vi "To CSV File.vi"(8 "error in (no error)":errorcluster, 9 "Path":path, 10 "engine configuration":refnum<class "engine configuration.lvclass">, 11 "PID Module editor node in":refnum<class "PID Module editor node.lvclass">) -> (0 "error out":errorcluster, 3 "PID Module editor node out":refnum<class "PID Module editor node.lvclass">)   [LabVIEW 2015, in "PID Module editor node.lvclass"]
uses:
  PID Module editor node.lvclass
  <vilib>/NI/Module Execution Interface/Engine Configuration/engine configuration.lvclass
  module/configuration/PID Module configuration.lvclass
  <vilib>/NI/Configuration Framework/serializable configuration/NISE_CEF_serializable configuration.lvclass/NISE_CEF_serializable configuration.ctl
  module/configuration/PID Module configuration.lvclass/PID Module configuration.ctl
  <vilib>/Utility/LVClass/Get LV Class Name.vi
  <vilib>/NI/Configuration Framework/error generator/NISE_error generator.vi
  <vilib>/NI/Tag Bus Module Framework/channel/TBM channel.lvclass
  <vilib>/NI/Configuration Framework/serializable configuration/NISE_CEF_serializable configuration.lvclass
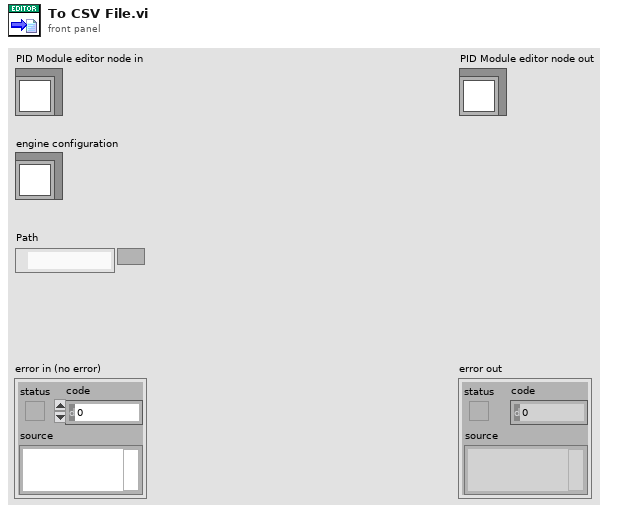
[diagram p1: front panel]
types:
  T1 = typedef "PID Module configuration.lvclass/Line.ctl" = cluster{"PID ID":string, "Setpoint":refnum<class "TBM channel.lvclass">, "Variable":refnum<class "TBM channel.lvclass">, "Output":refnum<class "TBM channel.lvclass">, "Output High":refnum<class "TBM channel.lvclass">, "Output Low":refnum<class "TBM channel.lvclass">, "P":refnum<class "TBM channel.lvclass">, "I":refnum<class "TBM channel.lvclass">, "D":refnum<class "TBM channel.lvclass">}
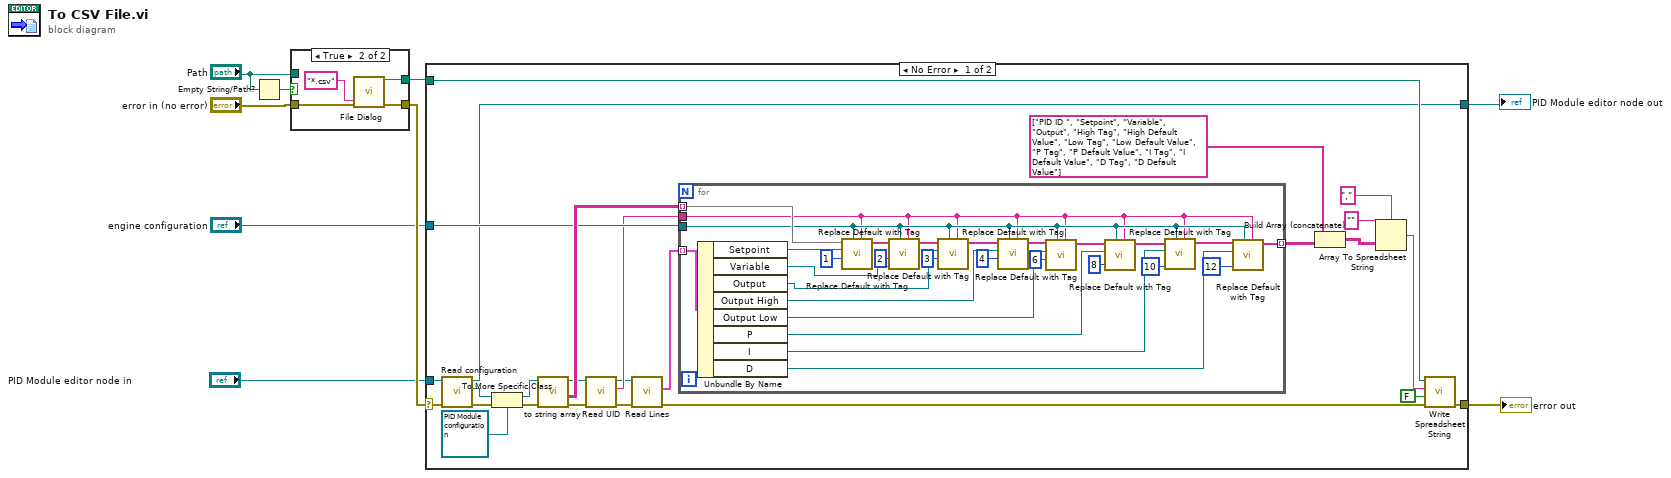
[diagram p0: block diagram]
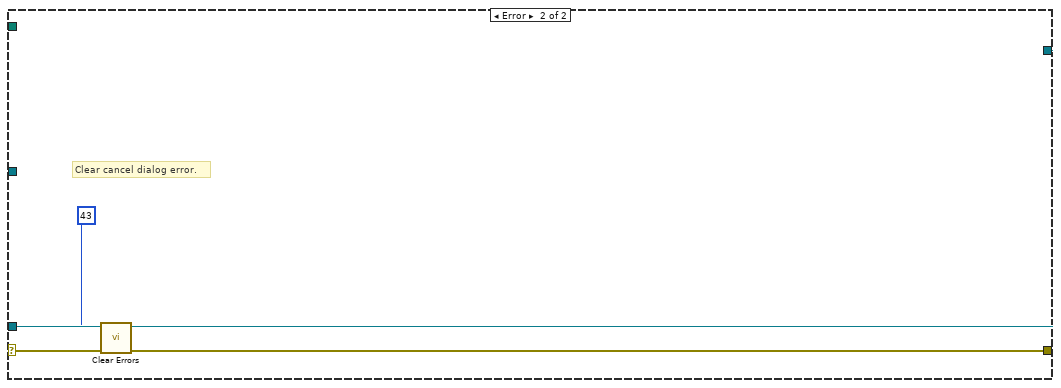
[diagram p3: hidden frame]
diagram:
  n1 = Empty String/Path?(string/path="Path") -> (empty?=w9:bool)
  n2 = case shown="True" w9 {
    tunnel: "error in (no error)" -> [w10 w14]
    tunnel: [w10 w13] -> w7
    tunnel: [w11 w12] -> w8
    tunnel: "Path" -> [w11 _]
    frame False {
    }
    frame True {
      n3 = call "File Dialog"("error in"=w14, "pattern (all files)"="*.csv") -> ("selected path"=w12:path, "error out"=w13:errorcluster)  [unwired: 10 in, 2 out]
    }
  }
  n4 = case shown="No Error" w7 {
    selector: w7 -> [w28 w72]
    tunnel: [w39 w71] -> w2
    tunnel: [w27 w73] -> w1
    tunnel: "PID Module editor node in" -> [w29 w73]
    tunnel: w8 -> [w35 _]
    tunnel: "engine configuration" -> [w32 _]
    frame No Error {
      n5 = call-dynamic "Read configuration.vi"("error in"=w28, "PID Module editor node in"=w29) -> ("error out"=w26:errorcluster, "configuration"=w25:refnum<class "NISE_CEF_serializable configuration.lvclass">, "PID Module editor node out"=w27:refnum<class "PID Module editor node.lvclass">)  [unwired: 7 in]
      n6 = To More Specific Class(target class=refnum<class "PID Module configuration.lvclass"> refnum ("tag bus configurable plugin module configuration"), reference=w25, error in=w26) -> (specific class reference=w41:refnum<class "PID Module configuration.lvclass">, error out=w40:errorcluster)
      n7 = call-dynamic "to string array.vi"("error in (no error)"=w40, "PID Module configuration in"=w41) -> ("error out"=w23:errorcluster, "Array"=w34:string[][], "PID Module configuration out"=w24:refnum<class "PID Module configuration.lvclass">)  [unwired: 6 in, 1 out]
      n8 = call <vilib>:"Read UID.vi"("error in"=w23, "configuration in"=w24) -> ("error out"=w21:errorcluster, "instance id"=w31:string, "configuration out"=w18:refnum<class "PID Module configuration.lvclass">)  [unwired: 7 in]
      n9 = call "Read Lines.vi"("error in (no error)"=w21, "PID Module configuration in"=w18) -> ("error out"=w20:errorcluster, "Lines"=w19:T1[])  [unwired: 7 in, 1 out]
      n10 = for {
        tunnel: w34 -> [w68] mode=indexing
        tunnel: [w56] -> w33 mode=indexing
        tunnel: w19 -> [w69] mode=indexing
        tunnel: w32 -> [w53]
        tunnel: w31 -> [w42]
        n11 = Unbundle By Name(w69) -> ("Setpoint"=w64:refnum<class "TBM channel.lvclass">, "Variable"=w63:refnum<class "TBM channel.lvclass">, "Output"=w62:refnum<class "TBM channel.lvclass">, "Output High"=w61:refnum<class "TBM channel.lvclass">, "Output Low"=w60:refnum<class "TBM channel.lvclass">, "P"=w59:refnum<class "TBM channel.lvclass">, "I"=w55:refnum<class "TBM channel.lvclass">, "D"=w54:refnum<class "TBM channel.lvclass">)
        n12 = call "Replace Default with Tag.vi"("instance id"=w42, "engine configuration in"=w53, "Channel Index"=1, "Channel"=w64, "Array in"=w68) -> ("Array out"=w52:string[])  [unwired: 6 in]
        n13 = call "Replace Default with Tag.vi"("instance id"=w42, "engine configuration in"=w53, "Channel Index"=2, "Channel"=w63, "Array in"=w52) -> ("Array out"=w67:string[])  [unwired: 6 in]
        n14 = call "Replace Default with Tag.vi"("instance id"=w42, "engine configuration in"=w53, "Channel Index"=3, "Channel"=w62, "Array in"=w67) -> ("Array out"=w51:string[])  [unwired: 6 in]
        n15 = call "Replace Default with Tag.vi"("instance id"=w42, "engine configuration in"=w53, "Channel Index"=4, "Channel"=w61, "Array in"=w51) -> ("Array out"=w66:string[])  [unwired: 6 in]
        n16 = call "Replace Default with Tag.vi"("instance id"=w42, "engine configuration in"=w53, "Channel Index"=6, "Channel"=w60, "Array in"=w66) -> ("Array out"=w65:string[])  [unwired: 6 in]
        n17 = call "Replace Default with Tag.vi"("instance id"=w42, "engine configuration in"=w53, "Channel Index"=8, "Channel"=w59, "Array in"=w65) -> ("Array out"=w58:string[])  [unwired: 6 in]
        n18 = call "Replace Default with Tag.vi"("instance id"=w42, "engine configuration in"=w53, "Channel Index"=10, "Channel"=w55, "Array in"=w58) -> ("Array out"=w57:string[])  [unwired: 6 in]
        n19 = call "Replace Default with Tag.vi"("instance id"=w42, "engine configuration in"=w53, "Channel Index"=12, "Channel"=w54, "Array in"=w57) -> ("Array out"=w56:string[])  [unwired: 6 in]
      }
      n20 = Build Array (concatenate)(string[] ["PID ID ", "Setpoint", "Variable", "Output", "High Tag", "High Default Value", "Low Tag", "Low Default Value", "P Tag", "P Default Value", "I Tag", "I Default Value", "D Tag", "D Default Value"] ("element"), w33) -> (w17:string[][])
      n21 = Array To Spreadsheet String(delimiter (Tab)=",", array=w17, 3:"" ("format string")) -> (spreadsheet string=w38:string)
      n22 = call <vilib>:"Write Spreadsheet String.vi"("error in"=w20, "append to file? (new file:F)"=FALSE, "spreadsheet string"=w38, "file path (dialog if empty)"=w35) -> ("error out"=w39:errorcluster)  [unwired: 6 in, 1 out]
    }
    frame Error {
      # "Clear cancel dialog error."
      n23 = call <vilib>:"Clear Errors.vi"("error in (no error)"=w72, "specific error code to clear (0: all)"=43) -> ("error out"=w71:errorcluster)  [unwired: 4 in, 1 out]
    }
  }
  "error out" <- w2
  "PID Module editor node out" <- w1
